vi "Adjust Register Order.vi"(7 "Order":T1, 11 "Register Values in":u16[](array[numeric]) format="%.0x") -> (3 "Register Values out":u16[](array[numeric]) format="%.0x")   [LabVIEW 2026, in "Modbus.lvlib" / "Modbus.lvclass"]
uses:
  Modbus.lvclass
  Types/Order.ctl
  Modbus.lvclass/Modbus.ctl
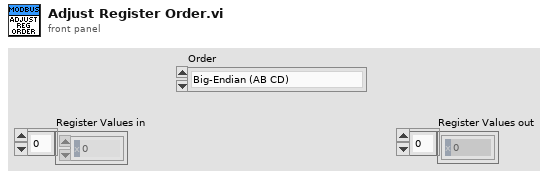
[diagram p1: front panel]
types:
  T1 = typedef "Modbus.lvlib/Modbus.lvclass/Order.ctl" = enum16{"Big-Endian (AB CD)", "Word-Swap (CD AB)", "Byte-Swap (BA DC)", "Little-Endian (DC BA)"}
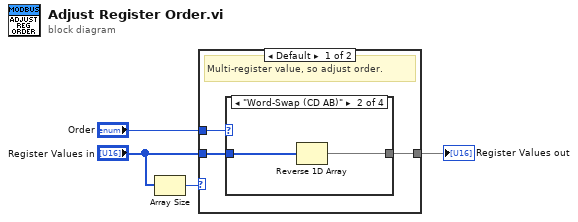
[diagram p0: block diagram]
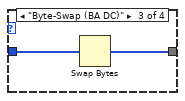
[diagram p3: hidden frame]
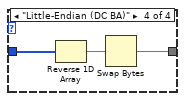
[diagram p4: hidden frame]
diagram:
  n1 = Array Size(array="Register Values in") -> (size(s)=w1:i32)
  n2 = case shown="Default" w1 {
    tunnel: "Register Values in" -> [w5 w16]
    tunnel: [w6 w16] -> w3
    tunnel: "Order" -> [w7 _]
    frame Default {
      # "Multi-register value, so adjust order."
      n3 = case shown="\"Word-Swap (CD AB)\"" w7 {
        tunnel: [w8 w9 w11 w13] -> w6
        tunnel: w5 -> [w8 w10 w12 w15]
        frame "Big-Endian (AB CD)" {
        }
        frame "Word-Swap (CD AB)" {
          n4 = Reverse 1D Array(array=w10) -> (reversed array=w9:u16[])
        }
        frame "Byte-Swap (BA DC)" {
          n5 = Swap Bytes(anything=w12) -> (byte swapped=w11:u16[])
        }
        frame "Little-Endian (DC BA)" {
          n6 = Reverse 1D Array(array=w15) -> (reversed array=w14:u16[])
          n7 = Swap Bytes(anything=w14) -> (byte swapped=w13:u16[])
        }
      }
    }
    frame 1 {
      # "Modbus standard defines Big-Endian order for single register values, so just pass through."
    }
  }
  "Register Values out" <- w3
